vi "Get TipText.vi"(8 "error in (no error)":errorcluster, 11 "object in":refnum<class "Button.lvclass">) -> (0 "error out":errorcluster, 2 "TipText":string, 3 "object out":refnum<class "Button.lvclass">)   [LabVIEW 2012, in "Button.lvclass"]
uses:
  Button.lvclass
  Button.lvclass/Button.ctl
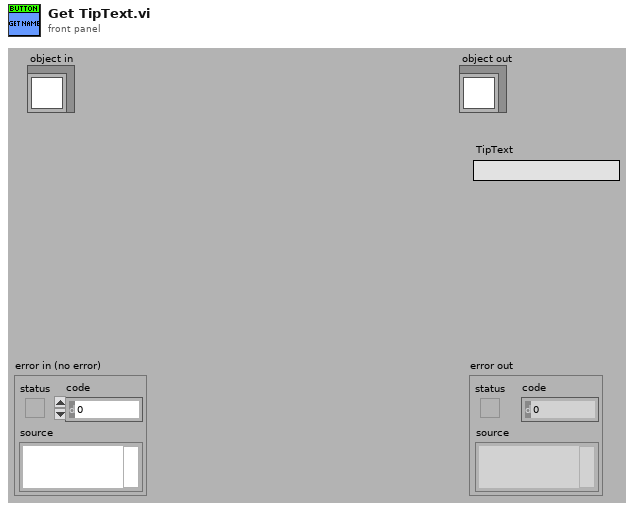
[diagram p1: front panel]
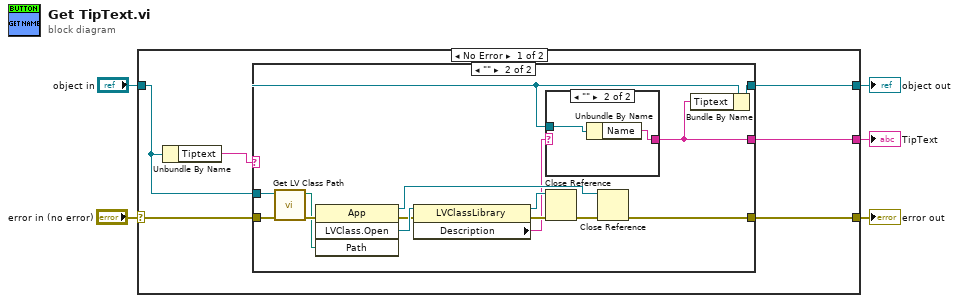
[diagram p0: block diagram]
diagram:
  n1 = case shown="No Error" "error in (no error)" {
    selector: "error in (no error)" -> [w10 w33]
    tunnel: [w9 w33] -> w4
    tunnel: [w6 w32] -> w2
    tunnel: "object in" -> [w8 w32]
    tunnel: [w11 _] -> w1
    frame No Error {
      n2 = Unbundle By Name(w8) -> ("Tiptext"=w7:string)
      n3 = case shown="\"\"" w7 {
        selector: w7 -> [w14 _]
        tunnel: [w14 w15] -> w11
        tunnel: w10 -> [w13 w19]
        tunnel: [w13 w18] -> w9
        tunnel: w8 -> [w12 w17]
        tunnel: [w12 w16] -> w6
        frame "False", Default {
        }
        frame "" {
          n4 = call <vilib>:"Get LV Class Path.vi"("error in (no error)"=w19, "object"=w17) -> ("error out"=w28:errorcluster, "class path"=w27:path)  [unwired: 8 in]
          n5 = invoke class="App" method="LVClass.Open"(error in=w28, "Path"=w27) -> (reference out=w21:refnum<vi>, error out=w25:errorcluster, "LVClass.Open"=w26:refnum<vi>)  [unwired: 2 in, 1 out]
          n6 = property class="LVClassLibrary"(reference=w26, error in=w25) -> (reference out=w23:refnum<vi>, error out=w24:errorcluster, "Description"=w20:string)
          n7 = case shown="\"\"" w20 {
            selector: w20 -> [w29 _]
            tunnel: [w29 w31] -> w15
            tunnel: w17 -> [_ w30]
            frame "False", Default {
            }
            frame "" {
              n8 = Unbundle By Name(w30) -> ("Name"=w31:string)
            }
          }
          n9 = Close Reference(reference=w23, error in (no error)=w24) -> (error out=w22:errorcluster)
          n10 = Close Reference(reference=w21, error in (no error)=w22) -> (error out=w18:errorcluster)
          n11 = Bundle By Name(cluster=w17, "Tiptext"=w15) -> (w16:refnum<class "Button.lvclass">)
        }
      }
    }
    frame Error {
    }
  }
  "error out" <- w4
  "object out" <- w2
  "TipText" <- w1
